vi "GMAP_API_CreateMapRef (SubVI).vi"(11 "Gmaps API key":string) -> (0 "error out":errorcluster, 3 "map file path":path)   [LabVIEW 2025]
doc: "This VI creates a reference to an HTML file,\ncontaining Google map, that is used by other API functions"
panel:
  # "This VI creates a reference to an HTML file,\ncontaining Google map, that is used by other API functions\nIn order to run a VI, you need to get Google maps API demo key"
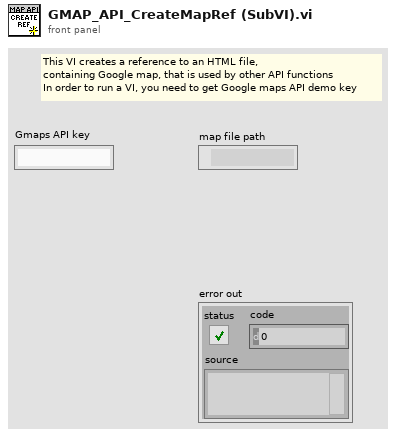
[diagram p1: front panel]
types:
  T1 = enum16{"open", "replace", "create", "open or create", "replace or create", "replace or create with confirmation"}
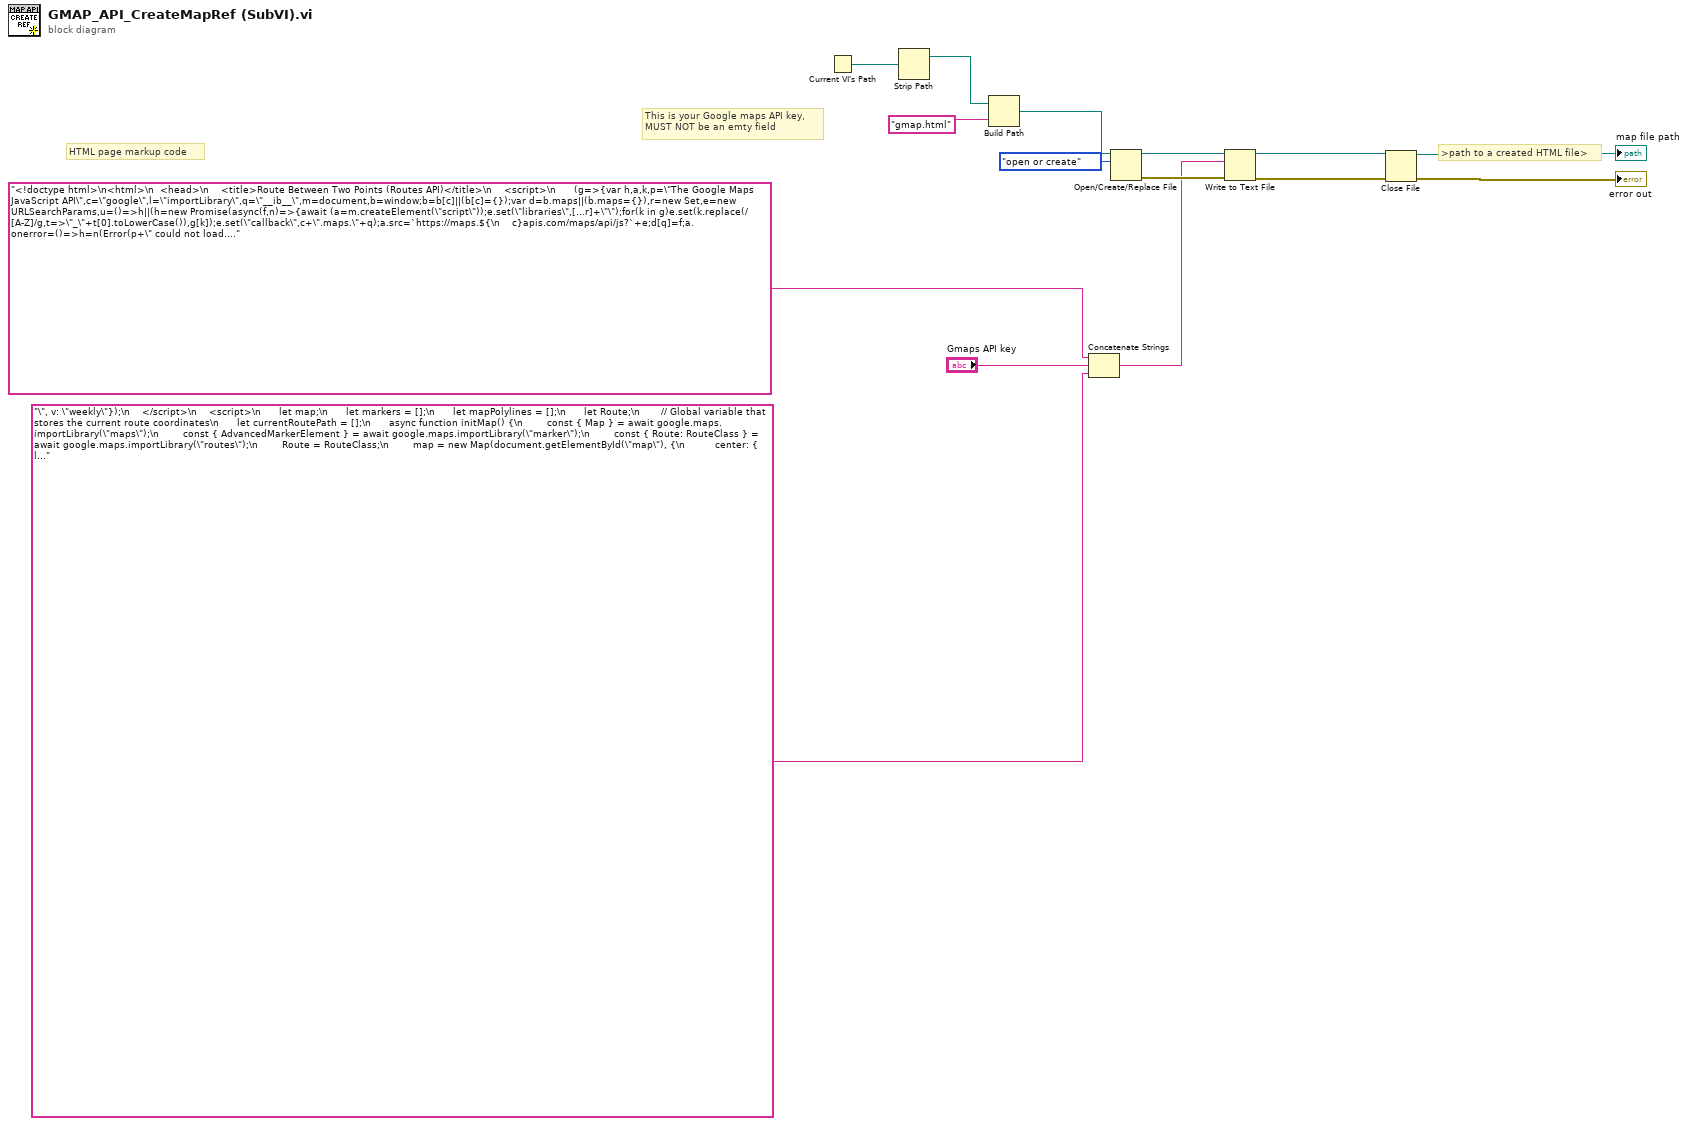
[diagram p0: block diagram]
diagram:
  # "HTML page markup code"
  # "This is your Google maps API key,\nMUST NOT be an emty field"
  # ">path to a created HTML file>"
  n1 = Current VI's Path() -> (path=w15:path)
  n2 = Strip Path(path=w15) -> (stripped path=w14:path)  [unwired: 1 out]
  n3 = Build Path(base path=w14, name or relative path="gmap.html") -> (appended path=w12:path)
  n4 = Concatenate Strings("<!doctype html>\n<html>\n  <head>\n    <title>Route Between Two Points (Routes API)</title>\n    <script>\n      (g=>{var h,a,k,p=\"The Google Maps JavaScript API\",c=\"google\",l=\"importLibrary\",q=\"__ib__\",m=document,b=window;b=b[c]||(b[c]={});var d=b.maps||(b.maps={}),r=new Set,e=new URLSearchParams,u=()=>h||(h=new Promise(async(f,n)=>{await (a=m.createElement(\"script\"));e.set(\"libraries\",[...r]+\"\");for(k in g)e.set(k.replace(/[A-Z]/g,t=>\"_\"+t[0].toLowerCase()),g[k]);e.set(\"callback\",c+\".maps.\"+q);a.src=`https://maps.${\n    c}apis.com/maps/api/js?`+e;d[q]=f;a.onerror=()=>h=n(Error(p+\" could not load.\"));a.nonce=m.querySelector(\"script[nonce]\")?.nonce||\"\";m.head.append(a)}));d[l]?console.warn(p+\" only loads once. Ignoring:\",g):d[l]=(f,...n)=>r.add(f)&&u().then(()=>d[l](f,...n))})\n      ({key: \"", "Gmaps API key", "\", v: \"weekly\"});\n    </script>\n    <script>\n      let map;\n      let markers = [];\n      let mapPolylines = [];\n      let Route;\n       // Global variable that stores the current route coordinates\n      let currentRoutePath = [];\n      async function initMap() {\n        const { Map } = await google.maps.importLibrary(\"maps\");\n        const { AdvancedMarkerElement } = await google.maps.importLibrary(\"marker\");\n        const { Route: RouteClass } = await google.maps.importLibrary(\"routes\");\n        Route = RouteClass;\n        map = new Map(document.getElementById(\"map\"), {\n          center: { lat: 30.291622, lng: -97.722012 },\n          zoom: 12,\n          mapId: \"DEMO_MAP_ID\",\n        });\n\t\t\n\t\t        map.addListener(\"click\", (event) => {\n          addMarker(event.latLng, AdvancedMarkerElement);\n          if (markers.length === 2) {\n            drawRoute(markers[0].position, markers[1].position);\n          }\n        });\n      }\n      function addMarker(location, AdvancedMarkerElement) {\n        if (markers.length === 2) {\n          markers.forEach((m) => (m.map = null));\n          markers = [];\n          mapPolylines.forEach((line) => line.setMap(null));\n          mapPolylines = [];\n          currentRoutePath = []; // Reset the stored path\n        }\n\n        const marker = new AdvancedMarkerElement({\n          map: map,\n          position: location,\n          title: markers.length === 0 ? \"Origin\" : \"Destination\",\n        });\n        markers.push(marker);\n      }\n\n      async function drawRoute(origin, destination) {\n        mapPolylines.forEach((line) => line.setMap(null));\n        mapPolylines = [];\n        currentRoutePath = [];\n\n        const request = {\n          origin: origin,\n          destination: destination,\n          travelMode: 'DRIVING',\n          fields: ['path', 'viewport'],\n        };\n        try {\n          const { routes } = await Route.computeRoutes(request);\n\n          if (!routes || routes.length === 0) {\n            console.warn('No routes found.');\n            return;\n          }\n          const route = routes[0];\n          currentRoutePath = route.path;\n          console.log('Route coordinates stored:', currentRoutePath.length, 'points');\n          // Draw the route on the map\n          mapPolylines = route.createPolylines();\n          mapPolylines.forEach((polyline) => polyline.setMap(map));\n          if (route.viewport) {\n            map.fitBounds(route.viewport);\n          }\n        } catch (error) {\n          window.alert(\"Directions request failed: \" + error);\n        }\n      }\n       // GLOBAL FUNCTION FOR LABVIEW\n      // Call this via InvokeScript(\"getRouteCoordinates\")\n      function getRouteCoordinates() {\n        // Convert LatLngAltitude objects to plain objects\n        const plainArray = currentRoutePath.map((point) => ({\n          lat: point.lat,\n          lng: point.lng,\n        }));\n        return JSON.stringify(plainArray);\n      }\n      function getRoutePointCount() {\n        return currentRoutePath.length;\n      }\n      function hasRoute() {\n        return currentRoutePath.length > 0;\n      }\n\n      initMap();\n    </script>\n    <style>\n      #map { height: 100%; }\n      html, body { height: 100%; margin: 0; padding: 0; }\n    </style>\n  </head>\n  <body>\n    <div id=\"map\"></div>\n  </body>\n</html>") -> (w2:string)
  n5 = Open/Create/Replace File(file path (use dialog)=w12, operation (0:open)=T1."open or create") -> (refnum out=w9:refnum<file>, error out=w10:errorcluster)  [unwired: 4 in, 1 out]
  n6 = Write to Text File(file (use dialog)=w9, text=w2, error in=w10) -> (refnum out=w6:refnum<file>, error out=w8:errorcluster)  [unwired: 1 in, 1 out]
  n7 = Close File(refnum=w6, error in=w8) -> (path=→"map file path":path, error out=→"error out":errorcluster)
